vi "Measurement Logic.vi"() -> ()   [LabVIEW 2025, in "DAQ_FiniteAI.lvlib"]
uses:
  DAQ_FiniteAI.lvlib
  <vilib>/Plug-In SDKs/Measurements/Measure Call Context/Measure Call Context.lvclass
  Measurement Configuration.ctl
  Measurement Results.ctl
  <vilib>/DAQmx/create/channels.llb/DAQmx Create Channel (AI-Voltage-Basic).vi
  <vilib>/DAQmx/configure/timing.llb/DAQmx Timing (Sample Clock).vi
  <vilib>/DAQmx/miscellaneous.llb/DAQmx Fill In Error Info.vi
  <vilib>/DAQmx/configure/trigger.llb/DAQmx Start Trigger (Digital Edge).vi
  <vilib>/measure/matone.llb/Extract Single Tone Information 1 Chan.vi
  <vilib>/DAQmx/read.llb/DAQmx Read (Analog Wfm 1Chan NSamp).vi
  <resource>/objmgr/daqmx.rc
  <vilib>/measure/NI_MAPro.lvlib
  <vilib>/DAQmx/configure/trigger.llb/DAQmx Start Trigger (None).vi
panel:
  out "measurement results":T1={"Actual_Sample_Rate"=0.0, "dt"=0.0, "Y"=[], "detected_amplitude"=1000000.0, "detected_frequency"=1000000.0} {"detected_frequency" format="%.2p"; "detected_amplitude" format="%.2p"; "Y" format="%.2p"; "dt" format="%.2p"; "Actual_Sample_Rate" format="%.2p"}
  in  "measurement configuration":T2={"Physical_Channel"="Lorem ipsum dolor sit", "Min_Voltage"=1.2, "Max_Voltage"=32.0, "Sample_Rate"=1000000.0, "Number_of_Samples"=32, "Source"=enum."PXI_Trig0", "Edge"=64} {"Edge" items=["Rising"=10280, "Falling"=10171]}
  out "measure call context out":refnum<class "Measure Call Context.lvclass">
  in  "measure call context in":refnum<class "Measure Call Context.lvclass">
  out "error out":errorcluster
  in  "error in":errorcluster
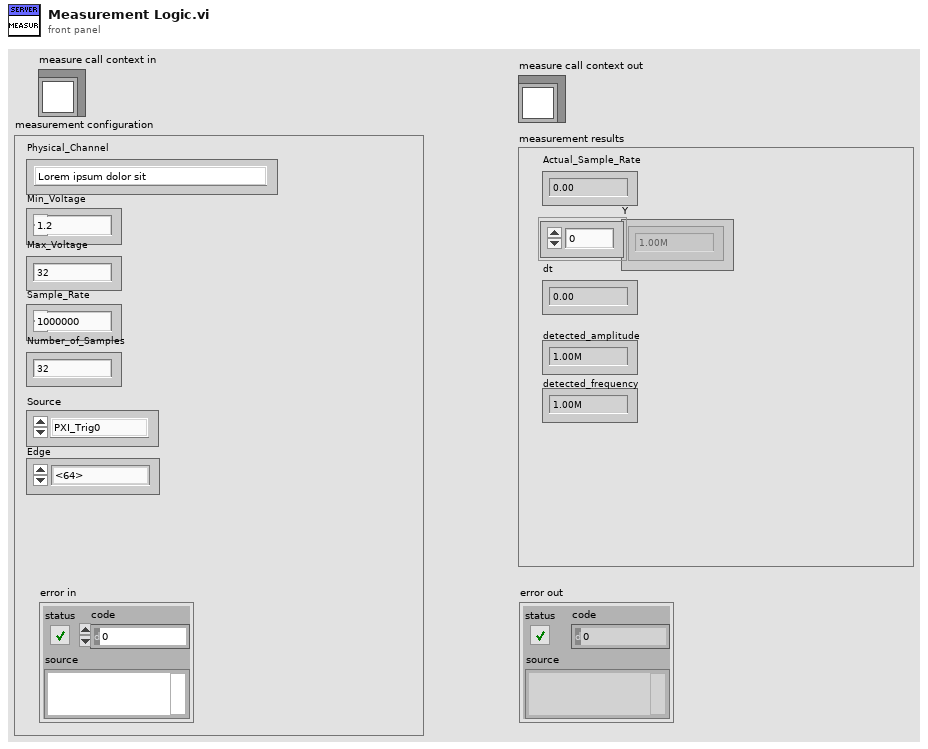
[diagram p1: front panel]
types:
  T1 = typedef "DAQ_FiniteAI.lvlib/Measurement Results.ctl" = cluster{"Actual_Sample_Rate":dbl, "dt":dbl, "Y":dbl[], "detected_amplitude":dbl, "detected_frequency":dbl}
  T2 = typedef "DAQ_FiniteAI.lvlib/Measurement Configuration.ctl" = cluster{"Physical_Channel":string, "Min_Voltage":dbl, "Max_Voltage":dbl, "Sample_Rate":dbl, "Number_of_Samples":i32, "Source":enum32{"NoTrigger", "PXI_Trig0", "PXI_Trig1", "PXI_Trig2", "PXI_Trig3", "PXI_Trig4", "PXI_Trig5", "PXI_Trig6", "PXI_Trig7"}, "Edge":i32}
  T3 = enum32{"NoTrigger", "PXI_Trig0", "PXI_Trig1", "PXI_Trig2", "PXI_Trig3", "PXI_Trig4", "PXI_Trig5", "PXI_Trig6", "PXI_Trig7"}
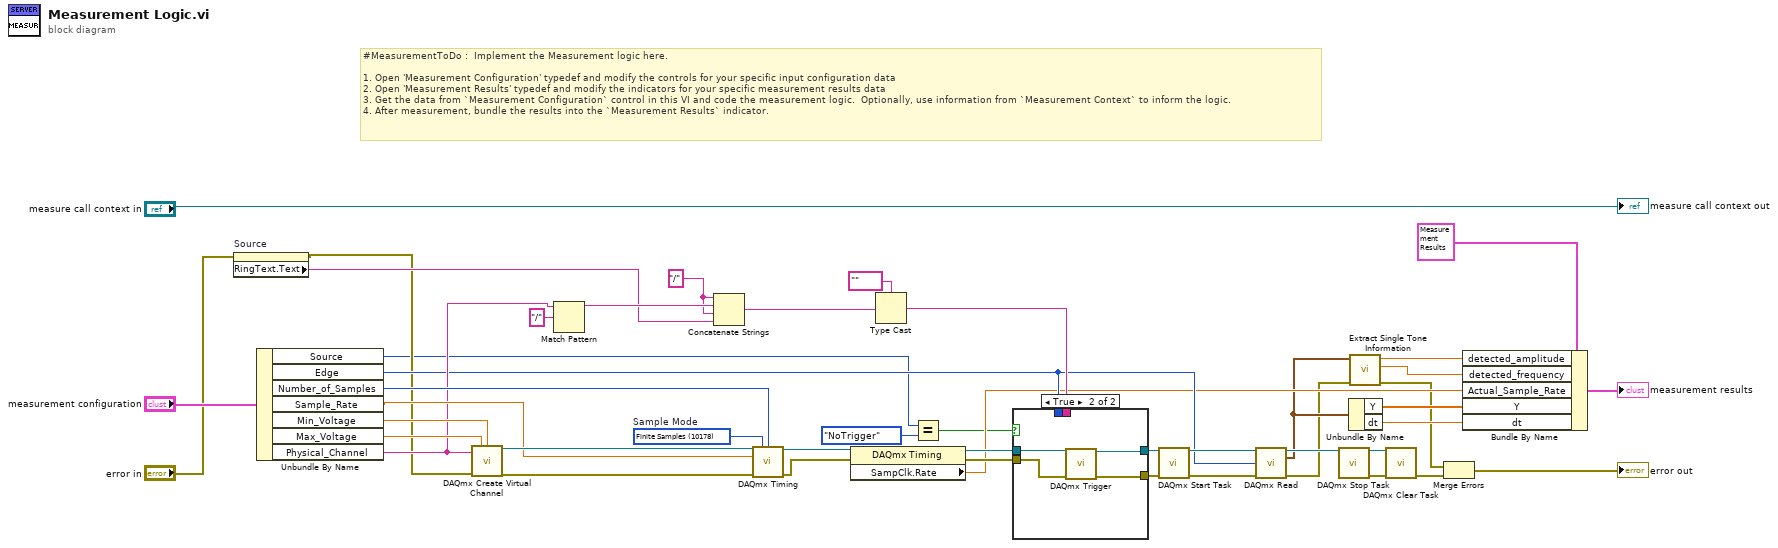
[diagram p0: block diagram]
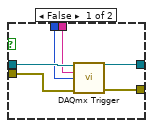
[diagram p2: hidden frame]
diagram:
  w14 = "/" ("string")
  w43 = 10178 items=["Finite Samples"=10178, "Continuous Samples"=10123, "Hardware Timed Single Point"=12522]  # Sample Mode
  # "#MeasurementToDo :  Implement the Measurement logic here.\n\n1. Open 'Measurement Configuration' typedef and modify the controls for your specific input configuration data\n2. Open 'Measurement Results' typedef and modify the indicators for your specific measurement results data\n3. Get the data from `Measurement Configuration` control in this VI and code the measurement logic.  Optionally, use information from `Measurement Context` to inform the logic.\n4. After measurement, bundle the results into the `Measurement Results` indicator."
  n1 = property on="Source" class="Enum (strict)"(error in="error in") -> (error out=w11:errorcluster, "RingText.Text"=w13:string)  [unwired: 1 in, 1 out]
  n2 = Unbundle By Name("measurement configuration") -> ("Source"=w3:T3, "Edge"=w21:i32, "Number_of_Samples"=w28:i32, "Sample_Rate"=w29:dbl, "Min_Voltage"=w30:dbl, "Max_Voltage"=w31:dbl, "Physical_Channel"=w27:string)
  n3 = call-poly <vilib>:"DAQmx Create Virtual Channel.vi"("maximum value"=w31, "minimum value"=w30, "physical channels"=w27, "error in"=w11) -> ("task out"=w41:refnum<k21>, "error out"=w42:errorcluster)  [unwired: 10 in]
  n4 = Match Pattern(string=w27, regular expression="/") -> (before substring=w25:string)  [unwired: 1 in, 3 out]
  n5 = Concatenate Strings(w14, w25, w14, w13) -> (w24:string)
  n6 = call-poly <vilib>:"DAQmx Timing.vi"("task/channels in"=w41, "sample mode"=w43, "samples per channel"=w28, "rate"=w29, "error in"=w42) -> ("task out"=w45:refnum<k21>, "error out"=w44:errorcluster)  [unwired: 9 in]
  n7 = property class="DAQmx Timing"(reference=w45, error in=w44) -> (reference out=w40:refnum<k21>, error out=w39:errorcluster, "SampClk.Rate"=w17:dbl)
  n8 = Type Cast(type=tag "" ("source"), x=w24) -> (*(type *) &x=w22:tag)
  n9 = Equal?(x=w3, y=T3."NoTrigger") -> (x = y?=w1:bool)
  n10 = case shown="True" w1 {
    tunnel: w40 -> [w52 w56]
    tunnel: w39 -> [w51 w55]
    tunnel: [w50 w53] -> w33
    tunnel: [w49 w54] -> w32
    tunnel: w22 -> [w48 _]
    tunnel: w21 -> [w47 _]
    frame False {
      n11 = call-poly <vilib>:"DAQmx Trigger.vi"("task/channels in"=w52, "source"=w48, "edge"=w47, "error in"=w51) -> ("task out"=w50:refnum<k21>, "error out"=w49:errorcluster)  [unwired: 10 in]
    }
    frame True {
      n12 = call-poly <vilib>:"DAQmx Trigger.vi"("task/channels in"=w56, "error in"=w55) -> ("task out"=w53:refnum<k21>, "error out"=w54:errorcluster)  [unwired: 12 in]
    }
  }
  n13 = call <vilib>:"DAQmx Start Task.vi"("task/channels in"=w33, "error in"=w32) -> ("task out"=w38:refnum<k21>, "error out"=w37:errorcluster)  [unwired: 12 in]
  n14 = call-poly <vilib>:"DAQmx Read.vi"("task/channels in"=w38, "number of samples per channel"=w21, "error in"=w37) -> ("task out"=w34:refnum<k21>, "data"=w10:waveform(dbl), "error out"=w7:errorcluster)  [unwired: 10 in]
  n15 = call <vilib>:"DAQmx Stop Task.vi"("task/channels in"=w34) -> ("task out"=w36:refnum<k21>, "error out"=w35:errorcluster)  [unwired: 13 in]
  n16 = Unbundle By Name(w10) -> ("Y"=w19:dbl[], "dt"=w18:dbl)
  n17 = call-poly <vilib>:"Extract Single Tone Information.vi"("error in (no error)"=w7, "time signal in"=w10) -> ("error out"=w5:errorcluster, "detected amplitude"=w8:dbl, "detected frequency"=w9:dbl)  [unwired: 4 in, 3 out]
  n18 = call <vilib>:"DAQmx Clear Task.vi"("task in"=w36, "error in"=w35) -> ("error out"=w6:errorcluster)  [unwired: 13 in]
  n19 = Merge Errors(w5, w6) -> (→"error out":errorcluster)
  n20 = Bundle By Name(cluster=T1 {"Actual_Sample_Rate"=0.0, "dt"=0.0, "Y"=[], "detected_amplitude"=1000000.0, "detected_frequency"=1000000.0} ("measurement results"), "detected_amplitude"=w9, "detected_frequency"=w8, "Actual_Sample_Rate"=w17, "Y"=w19, "dt"=w18) -> (→"measurement results":T1)
  "measure call context out" <- "measure call context in"
